vi "Parse DB.vi"(8 "error in (no error)":errorcluster, 11 "Path in":path=path "C:/work/SE/Opportunities/2012/Pilatus/201210/TestXMLs/Receiver.xml") -> (0 "error out":errorcluster, 3 "channels":T1)   [LabVIEW 2015, in "AIT 429 System Explorer.lvlib"]
uses:
  AIT 429 System Explorer.lvlib
  Controls/AIT_Channel Array.ctl
  Controls/AIT_Channel.ctl
  Controls/AIT_Label.ctl
  Controls/AIT_Word.ctl
  Controls/ARINCParam.ctl
  Shared/Controls and Global/TransferType.ctl
  <userlib>/ARINC-429/vi/enum/Owl429ChannelSpeed.ctl
  <userlib>/ARINC-429/Owl429.lvlib
  Shared/AIT 429 Shared.lvlib
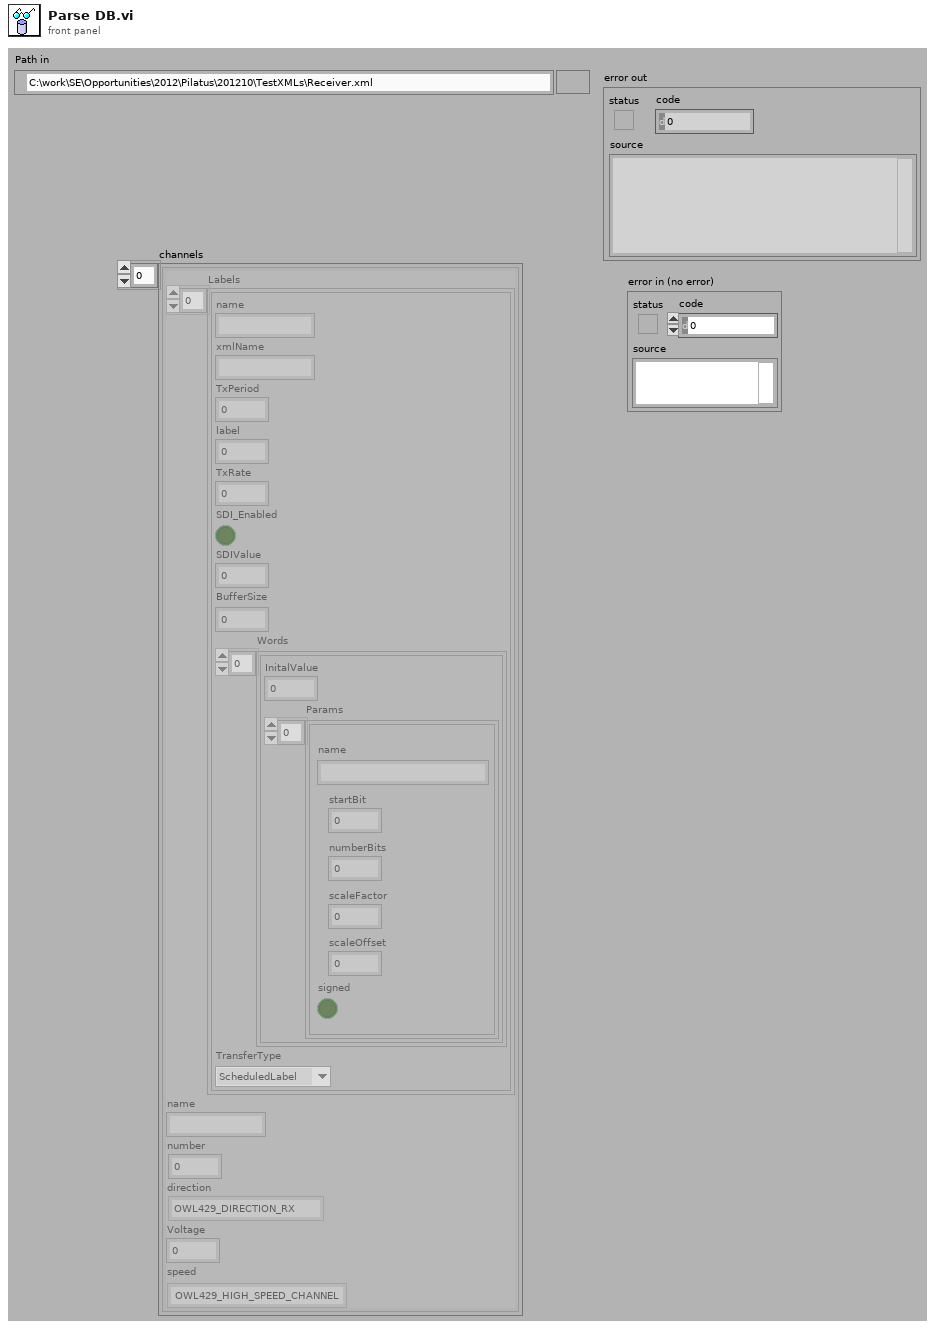
[diagram p1: front panel]
types:
  T1 = typedef "AIT 429 System Explorer.lvlib/AIT_Channel Array.ctl" = T2[]
  T2 = typedef "AIT 429 System Explorer.lvlib/AIT_Channel.ctl" = cluster{"Labels":T3[], "name":string, "number":u8, "direction":enum16{"OWL429_DIRECTION_RX", "OWL429_DIRECTION_TX"}, "Voltage":dbl, "speed":T7}
  T3 = typedef "AIT 429 System Explorer.lvlib/AIT_Label.ctl" = cluster{"name":string, "xmlName":string, "TxPeriod":u32, "label":u32, "TxRate":dbl, "SDI_Enabled":bool, "SDIValue":u8, "BufferSize":u32, "Words":T4[], "TransferType":T6}
  T4 = typedef "AIT 429 System Explorer.lvlib/AIT_Word.ctl" = cluster{"InitalValue":u32, "Params":T5[]}
  T5 = typedef "AIT 429 System Explorer.lvlib/ARINCParam.ctl" = cluster{"name":string, "startBit":i32, "numberBits":i32, "scaleFactor":dbl, "scaleOffset":dbl, "signed":bool}
  T6 = typedef "AIT 429 Shared.lvlib/TransferType.ctl" = enum16{"ScheduledLabel", "Acyclic", "Block", "Strobe"}
  T7 = typedef "Owl429.lvlib/Owl429ChannelSpeed.ctl" = enum16{"OWL429_HIGH_SPEED_CHANNEL", "OWL429_LOW_SPEED_CHANNEL"}
  T8 = typedef "AIT 429 System Explorer.lvlib/ChannelParams.ctl" = cluster{"ChannelNum":u8, "LabelParams":T9[], "direction":enum16{"OWL429_DIRECTION_RX", "OWL429_DIRECTION_TX"}}
  T9 = typedef "AIT 429 System Explorer.lvlib/LabelParam.ctl" = cluster{"LabelInfo":T10, "ARINCParams":T5[]}
  T10 = typedef "AIT 429 System Explorer.lvlib/LabelInfo.ctl" = cluster{"label":u32, "SDI_Enabled":bool, "SDI":u8}
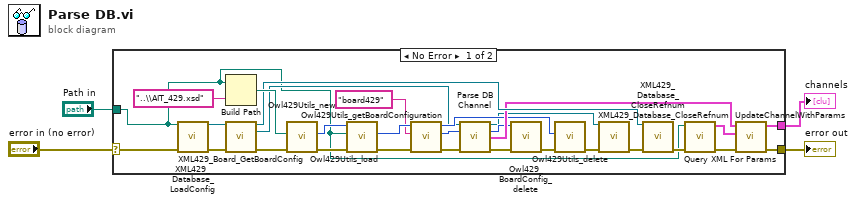
[diagram p0: block diagram]
diagram:
  n1 = case shown="No Error" "error in (no error)" {
    selector: "error in (no error)" -> [w33 w34]
    tunnel: "Path in" -> [w5 _]
    tunnel: [w19 w34] -> w2
    tunnel: [w20 _] -> w1
    frame No Error {
      n2 = call "XML429_Database_LoadConfig.vi"("FilePath"=w5, "Error in"=w33) -> ("ConfigHandle"=w32:refnum<k20>, "Error out"=w31:errorcluster)  [unwired: 12 in]
      n3 = Build Path(base path=w5, name or relative path="..\\AIT_429.xsd") -> (appended path=w28:path)
      n4 = call "XML429_Board_GetBoardConfig.vi"("ConfigHandle in"=w32, "Error in"=w31) -> ("ConfigHandle out"=w14:refnum<k20>, "BoardConfig"=w7:refnum<k20>, "Error out"=w29:errorcluster)  [unwired: 11 in]
      n5 = call <userlib>:"Owl429Utils_new.vi"("error in (no error)"=w29, "Xml Schema Path in"=w28) -> ("error out"=w27:errorcluster, "xml config handle"=w26:u32)  [unwired: 8 in]
      n6 = call <userlib>:"Owl429Utils_load.vi"("error in (no error)"=w27, "Path in"=w5, "xml config handle"=w26) -> ("error out"=w25:errorcluster, "xml config handle"=w24:u32)  [unwired: 7 in]
      n7 = call <userlib>:"Owl429Utils_getBoardConfiguration.vi"("error in (no error)"=w25, "X Path"="board429", "xml config handle"=w24) -> ("error out"=w13:errorcluster, "board config handle"=w8:u32, "xml config handle"=w9:u32)  [unwired: 6 in]
      n8 = call "Parse DB Channel.vi"("XMLBoardConfig in"=w7, "BoardConfigHandle in"=w8, "Error in"=w13) -> ("XMLBoardConfig out"=w6:refnum<k20>, "BoardConfigHandle out"=w10:u32, "Array"=w11:T2[], "Error out"=w12:errorcluster)  [unwired: 9 in]
      n9 = call <userlib>:"Owl429_BoardConfig_delete.vi"("error in (no error)"=w12, "config handle"=w10) -> ("error out"=w22:errorcluster)  [unwired: 9 in]
      n10 = call <userlib>:"Owl429Utils_delete.vi"("error in (no error)"=w22, "xml config handle"=w9) -> ("error out"=w15:errorcluster)  [unwired: 9 in]
      n11 = call "XML429_Database_CloseRefnum.vi"("XMLRefnum"=w6, "Error in"=w15) -> ("Error out"=w16:errorcluster)  [unwired: 13 in]
      n12 = call "XML429_Database_CloseRefnum.vi"("XMLRefnum"=w14, "Error in"=w16) -> ("Error out"=w21:errorcluster)  [unwired: 13 in]
      n13 = call "Query XML For Params.vi"("error in (no error)"=w21, "XML File Path"=w5) -> ("error out"=w18:errorcluster, "Array"=w17:T8[])  [unwired: 8 in]
      n14 = call "UpdateChannelWithParams.vi"("error in"=w18, "ParamArray"=w17, "channels in"=w11) -> ("error out"=w19:errorcluster, "channels out"=w20:T1)  [unwired: 7 in]
    }
    frame Error {
    }
  }
  "error out" <- w2
  "channels" <- w1
